vi "Update_Status_Bar.vi"(0 "State":string, 1 "Previous State":string, 5 "Table in":refnum<vi>, 7 "Debug?":bool, 11 "Error In":errorcluster, 12 "File Refnum":refnum<file>) -> (15 "Error Out":errorcluster)   [LabVIEW 2026, in "Core.lvlib"]
doc: "Updates the application status log by recording state transitions, updating the status table, and optionally writing debug information to a log file."
uses:
  Core.lvlib
  TypeDefs/Enum_Notifier_Name.ctl
  TypeDefs/Enum_Notifier_Options.ctl
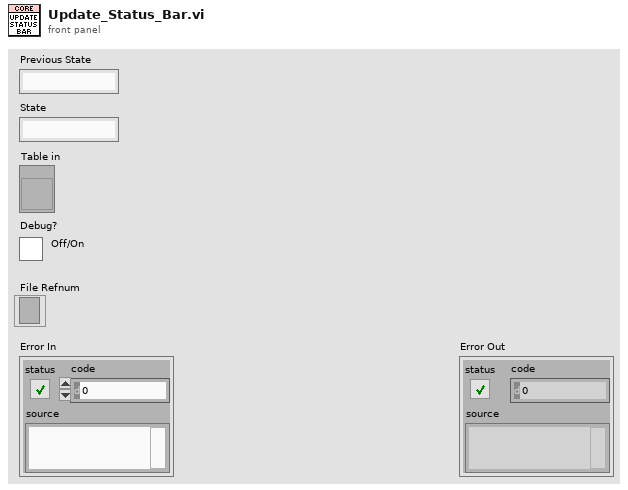
[diagram p1: front panel]
types:
  T1 = typedef "Core.lvlib/Enum_Notifier_Options.ctl" = enum16{"Create", "Send", "Status", "Release"}
  T2 = typedef "Core.lvlib/Enum_Notifier_Name.ctl" = enum16{"Device Type", "Test", "Instrument Spec", "Measurement Spec", "Status"}
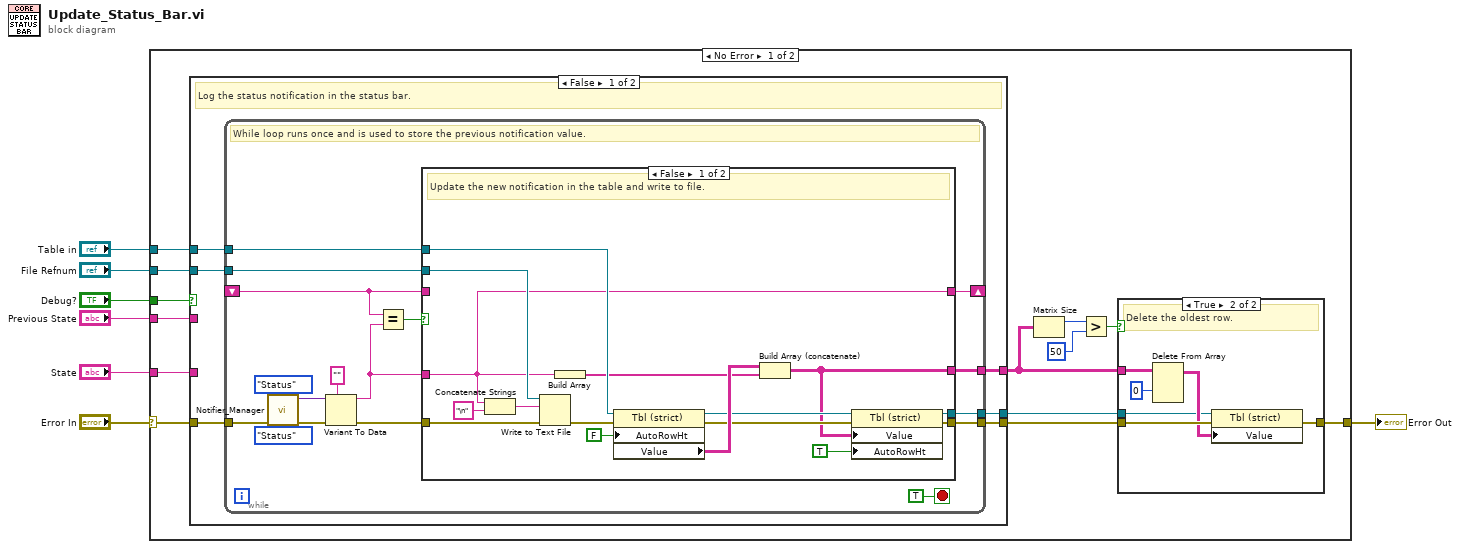
[diagram p0: block diagram]
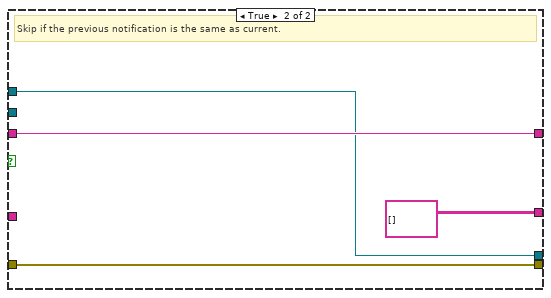
[diagram p3: hidden frame]
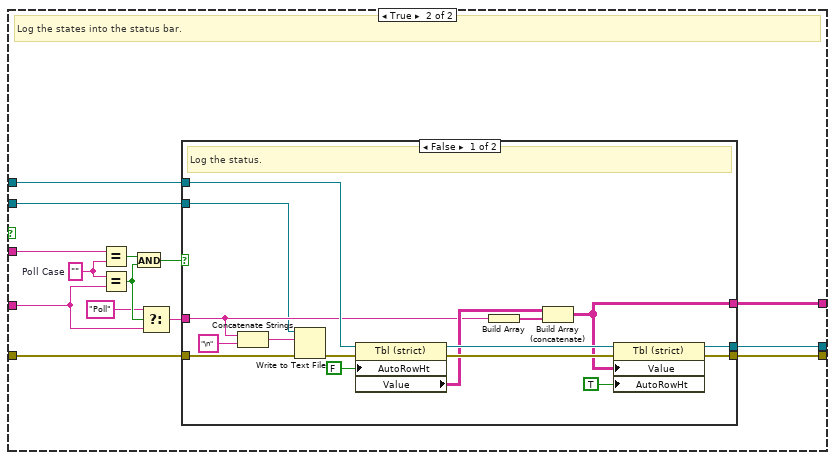
[diagram p4: hidden frame]
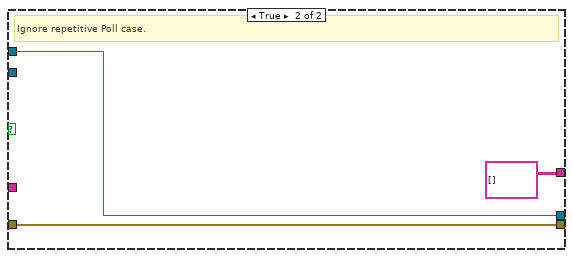
[diagram p5: hidden frame]
diagram:
  n1 = case shown="No Error" "Error In" {
    selector: "Error In" -> [w20 w104]
    tunnel: "Debug?" -> [w19 _]
    tunnel: "Table in" -> [w18 _]
    tunnel: [w14 w104] -> w4
    tunnel: "File Refnum" -> [w10 _]
    tunnel: "Previous State" -> [w9 _]
    tunnel: "State" -> [w8 _]
    frame No Error {
      n2 = case shown="False" w19 {
        tunnel: w20 -> [w33 w84]
        tunnel: w18 -> [w32 w83]
        tunnel: [w31 w82] -> w17
        tunnel: [w30 w78] -> w12
        tunnel: [w29 w77] -> w11
        tunnel: w10 -> [w28 w75]
        tunnel: w9 -> [_ w76]
        tunnel: w8 -> [_ w73]
        frame False {
          # "Log the status notification in the status bar."
          n3 = while {
            tunnel: w33 -> [w50]
            shift-right: [w42] -> _
            shift-left: _ -> [w41]
            tunnel: w32 -> [w39]
            tunnel: [w37] -> w31
            tunnel: [w36] -> w30
            tunnel: [w35] -> w29
            tunnel: w28 -> [w34]
            stop <- TRUE stop-if-true
            # "While loop runs once and is used to store the previous notification value."
            n4 = call "Notifier_Manager.vi"("Notifier Name"=Enum_Notifier_Name."Status", "Error In"=w50, "Notifier Options"=Enum_Notifier_Options."Status") -> ("Notifier Data"=w45:variant, "Error Out"=w47:errorcluster)  [unwired: 11 in]
            n5 = Variant To Data(error in=w47, type="", Variant=w45) -> (data=w38:string, error out=w40:errorcluster)
            n6 = Equal?(x=w41, y=w38) -> (x = y?=w43:bool)
            n7 = case shown="False" w43 {
              tunnel: [w54 w70] -> w42
              tunnel: w41 -> [_ w70]
              tunnel: w40 -> [w66 w69]
              tunnel: w39 -> [w64 w68]
              tunnel: w38 -> [w54 _]
              tunnel: [w61 w69] -> w37
              tunnel: [w60 w68] -> w36
              tunnel: [w57 string[][] [] ("Value")] -> w35
              tunnel: w34 -> [w55 _]
              frame False {
                # "Update the new notification in the table and write to file."
                n8 = Concatenate Strings(w54, "\n" ("string")) -> (w53:string)
                n9 = Write to Text File(file (use dialog)=w55, text=w53, error in=w66) -> (error out=w56:errorcluster)  [unwired: 1 in, 2 out]
                n10 = Build Array(w54) -> (w51:string[])
                n11 = property class="Tbl (strict)"(reference=w64, error in=w56, "AutoRowHt"=FALSE ("Autosizing Row Height")) -> (reference out=w59:refnum<vi>, error out=w62:errorcluster, "Value"=w63:string[][])
                n12 = Build Array (concatenate)(w63, w51) -> (w57:string[][])
                n13 = property class="Tbl (strict)"(reference=w59, error in=w62, "Value"=w57, "AutoRowHt"=TRUE ("Autosizing Row Height")) -> (reference out=w60:refnum<vi>, error out=w61:errorcluster)
              }
              frame True {
                # "Skip if the previous notification is the same as current."
              }
            }
          }
        }
        frame True {
          w81 = ""  # Poll Case
          # "Log the states into the status bar."
          n14 = Equal?(x=w76, y=w81) -> (x = y?=w80:bool)
          n15 = Equal?(x=w81, y=w73) -> (x = y?=w74:bool)
          n16 = And(x=w80, y=w74) -> (x .and. y?=w79:bool)
          n17 = Select(t="Poll", s=w74, f=w73) -> (s? t:f=w71:string)
          n18 = case shown="False" w79 {
            tunnel: w84 -> [w89 w103]
            tunnel: w83 -> [w100 w102]
            tunnel: [w98 w103] -> w82
            tunnel: w71 -> [w87 _]
            tunnel: [w93 w102] -> w78
            tunnel: [w92 string[][] [] ("Value")] -> w77
            tunnel: w75 -> [w86 _]
            frame False {
              # "Log the status."
              n19 = Concatenate Strings(w87, "\n" ("string")) -> (w91:string)
              n20 = Write to Text File(file (use dialog)=w86, text=w91, error in=w89) -> (error out=w88:errorcluster)  [unwired: 1 in, 2 out]
              n21 = property class="Tbl (strict)"(reference=w100, error in=w88, "AutoRowHt"=FALSE ("Autosizing Row Height")) -> (reference out=w97:refnum<vi>, error out=w99:errorcluster, "Value"=w96:string[][])
              n22 = Build Array(w87) -> (w85:string[])
              n23 = Build Array (concatenate)(w96, w85) -> (w92:string[][])
              n24 = property class="Tbl (strict)"(reference=w97, error in=w99, "Value"=w92, "AutoRowHt"=TRUE ("Autosizing Row Height")) -> (reference out=w93:refnum<vi>, error out=w98:errorcluster)
            }
            frame True {
              # "Ignore repetitive Poll case."
            }
          }
        }
      }
      n25 = Matrix Size(0:w11) -> (1:w16:i32)  [unwired: 1 out]
      n26 = Greater?(x=w16, y=50) -> (0:w13:bool)
      n27 = case shown="True" w13 {
        tunnel: w17 -> [w21 w27]
        tunnel: [w21 w23] -> w14
        tunnel: w11 -> [_ w26]
        tunnel: w12 -> [_ w24]
        frame False {
          # "Continue."
        }
        frame True {
          # "Delete the oldest row."
          n28 = Delete From Array(array=w26, index (row)=0) -> (array with subset deleted=w25:string[][])  [unwired: 2 in, 1 out]
          n29 = property class="Tbl (strict)"(reference=w24, error in=w27, "Value"=w25) -> (error out=w23:errorcluster)  [unwired: 1 out]
        }
      }
    }
    frame Error {
    }
  }
  "Error Out" <- w4
